vi "ECGsimulated.vi"() -> ()   [LabVIEW 2026]
panel:
  out "Peak to Peak":dbl
  out "Positive Peak":dbl
  out "data":dynamicdata(graph)
  in  "stop (F)":bool
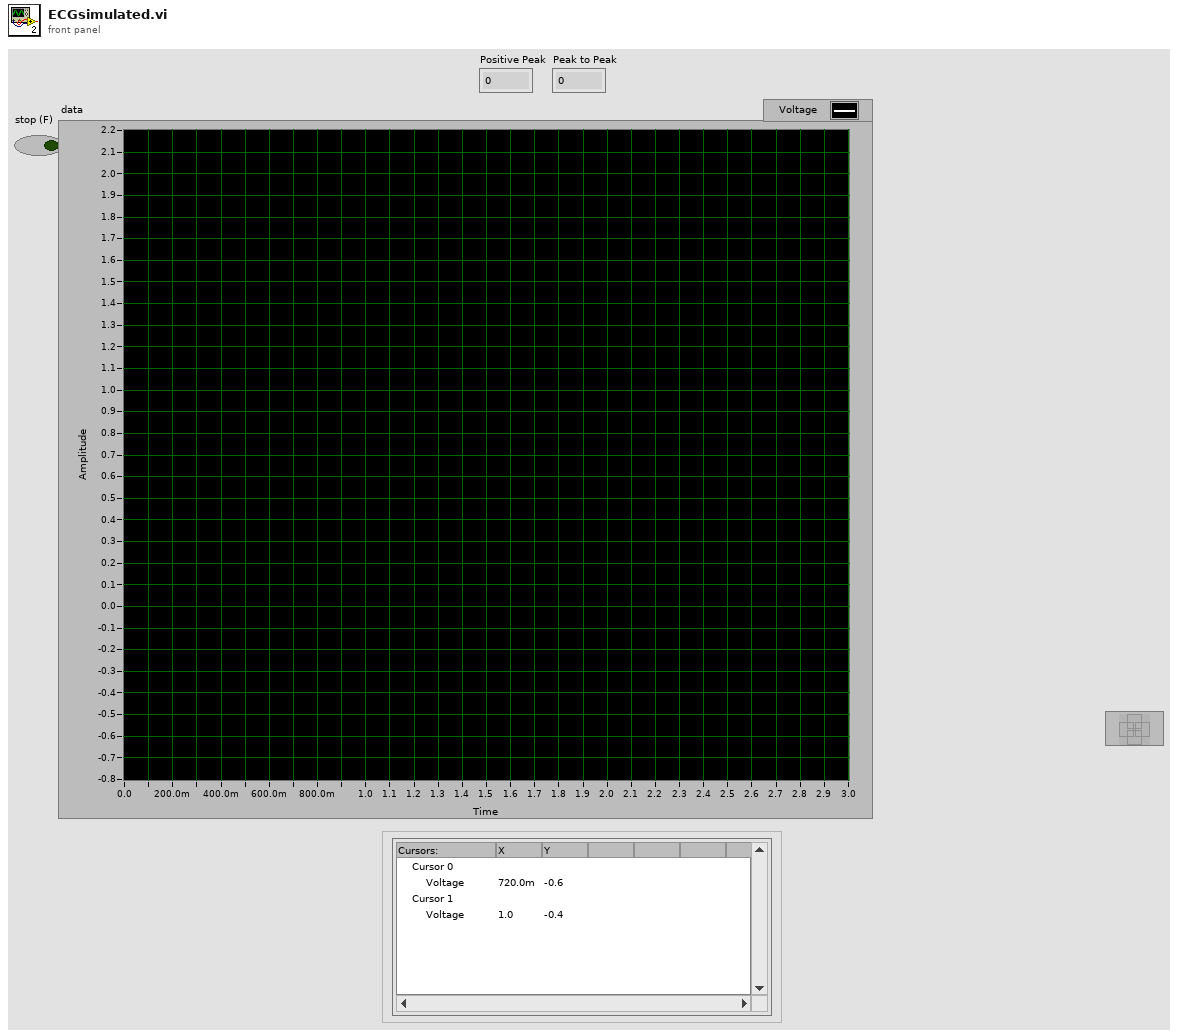
[diagram p1: front panel]
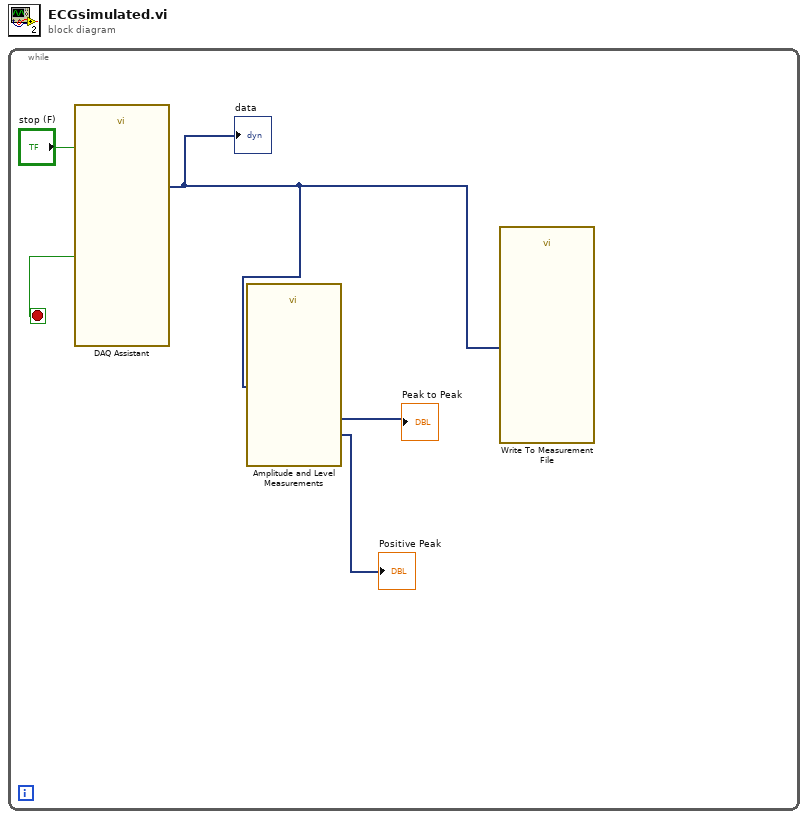
[diagram p0: block diagram]
diagram:
  n1 = while {
    stop <- w4 stop-if-true
    n2 = call "DAQ Assistant"("stop (F)"="stop (F)") -> ("data"=w3:dynamicdata, "stopped"=w4:bool)  [unwired: 15 in, 2 out]
    "data" <- w3
    n3 = call "Amplitude and Level Measurements"("Signals"=w3) -> ("Positive Peak"=→"Positive Peak":dynamicdata, "Peak to Peak"=→"Peak to Peak":dynamicdata)  [unwired: 10 in, 3 out]
    n4 = call "Write To Measurement File"("Signals"=w3) -> ()  [unwired: 16 in, 3 out]
  }
